vi "Add File.vi"(8 "error in":errorcluster, 9 "File Path":path, 10 "Whitelist constant":path, 11 "IHash Whitelist Handler in":refnum<class "IHash Whitelist Handler.lvclass">) -> (0 "error out":errorcluster, 3 "IHash Whitelist Handler out":refnum<class "IHash Whitelist Handler.lvclass">)   [LabVIEW 2026, in "IHash Whitelist Handler.lvclass"]
doc: "Add the hash of the provided file to the specified whitelist constant."
uses:
  IHash Whitelist Handler.lvclass
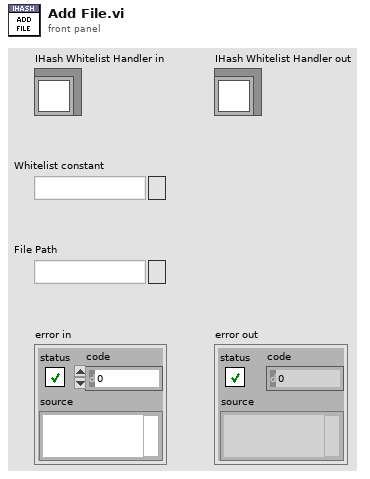
[diagram p1: front panel]
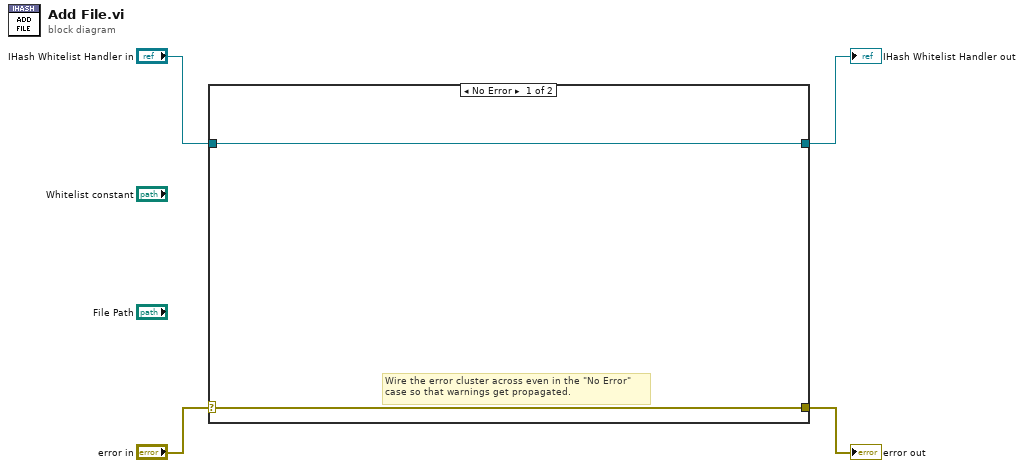
[diagram p0: block diagram]
diagram:
  n1 = case shown="No Error" "error in" {
    selector: "error in" -> [w6 w8]
    tunnel: [w6 w8] -> w3
    tunnel: [w5 w7] -> w1
    tunnel: "IHash Whitelist Handler in" -> [w5 w7]
    frame No Error {
      # "Wire the error cluster across even in the \"No Error\"\ncase so that warnings get propagated."
    }
    frame Error {
    }
  }
  "error out" <- w3
  "IHash Whitelist Handler out" <- w1
